vi "I2C Message Buffer - Destroy.vi"(8 "error in (no error)":errorcluster) -> (0 "error out":errorcluster)   [LabVIEW 2025, in "I2C Bus Monitor.lvclass"]
uses:
  I2C Bus Monitor.lvclass
  I2C Bus Monitor.lvclass/I2C Bus Monitor.ctl
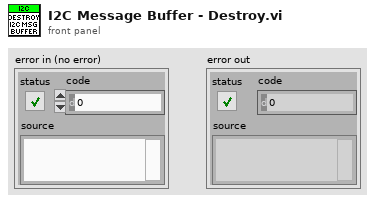
[diagram p1: front panel]
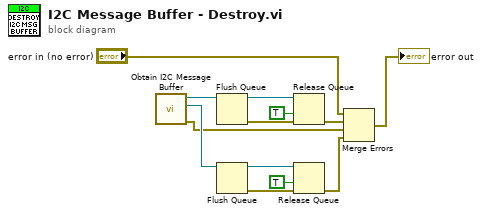
[diagram p0: block diagram]
diagram:
  n1 = call "Obtain I2C Message Buffer.vi"() -> ("error out"=w1:errorcluster, "Msgs per Txn Queue"=w2:refnum<queue>, "I2C Message Queue"=w3:refnum<queue>)  [unwired: 9 in]
  n2 = Flush Queue(queue=w3) -> (queue out=w10:refnum<queue>, error out=w11:errorcluster)  [unwired: 1 in, 1 out]
  n3 = Flush Queue(queue=w2) -> (queue out=w9:refnum<queue>, error out=w8:errorcluster)  [unwired: 1 in, 1 out]
  n4 = Release Queue(queue=w10, force destroy? (F)=TRUE, error in (no error)=w11) -> (error out=w13:errorcluster)  [unwired: 2 out]
  n5 = Release Queue(queue=w9, force destroy? (F)=TRUE, error in (no error)=w8) -> (error out=w5:errorcluster)  [unwired: 2 out]
  n6 = Merge Errors("error in (no error)", w13, w1, w5) -> (→"error out":errorcluster)
